vi "CP Profile selection_MS.vi"(8 "Signal Tag AZ":string[](array[string]), 11 "Long Signal Profile Table A":string[][](table) caption="Long Singla Profile Table") -> (3 "CP selected IDX":T1)   [LabVIEW 2018]
panel:
  out "M_MxRight_No":string[](array[string])
  out "M_RRead_Seq":string[](array[string])
  out "S# [n]":string[](array[string])
  out "L# [n]":string[](array[string])
  out "MSeq_ENo":string[](array[string])
  out "MSeq_SNo":string[](array[string])
  out "Later Seq":string[](array[string])
  out "Seq":string[](array[string])
  out "Front Seq":string[](array[string])
  out "Seq ENo":string[](array[string])
  out "Seq SNo":string[](array[string])
  out "Mx Right Read Seq":string[](array[string])
  out "Direction":string[](array[string])
  out "Assinged Sequence":string[](array[string])
  out "S CP IDX End [n]":string[](array[string])
  out "S CP IDX Start [n]":string[](array[string])
  out "サイズ":i32
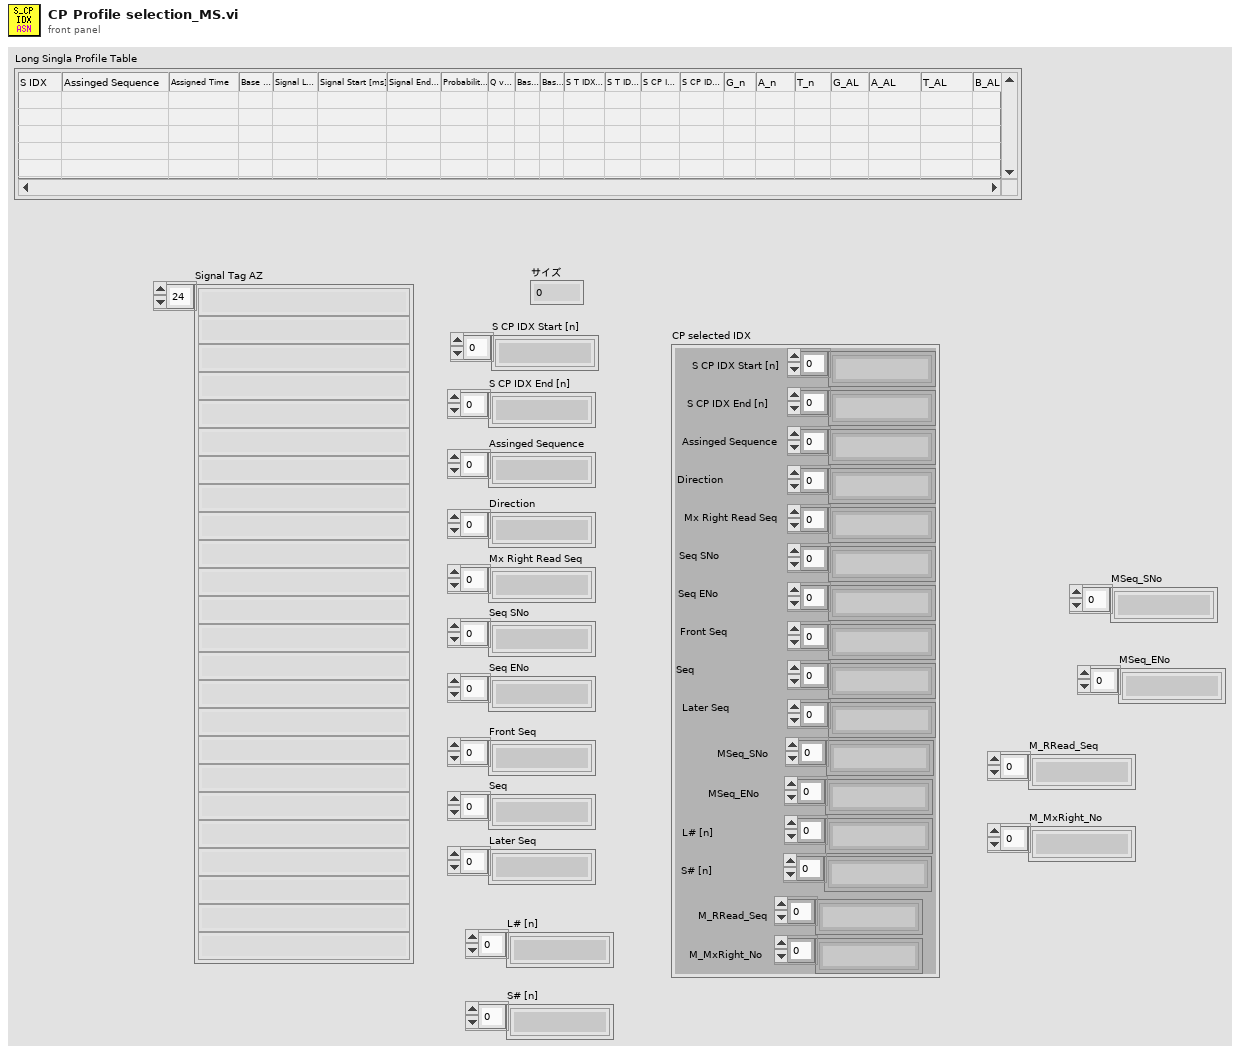
[diagram p1: front panel]
types:
  T1 = cluster{"S CP IDX Start [n]":string[], "S CP IDX End [n]":string[], "Assinged Sequence":string[], "Direction":string[], "Mx Right Read Seq":string[], "Seq SNo":string[], "Seq ENo":string[], "Front Seq":string[], "Seq":string[], "Later Seq":string[], "MSeq_SNo":string[], "MSeq_ENo":string[], "L# [n]":string[], "S# [n]":string[], "M_RRead_Seq":string[], "M_MxRight_No":string[]}
  T2 = cluster{string[], string[], string[], string[], string[], string[], string[], string[], string[], string[], string[], string[], string[], string[], string[], string[]}
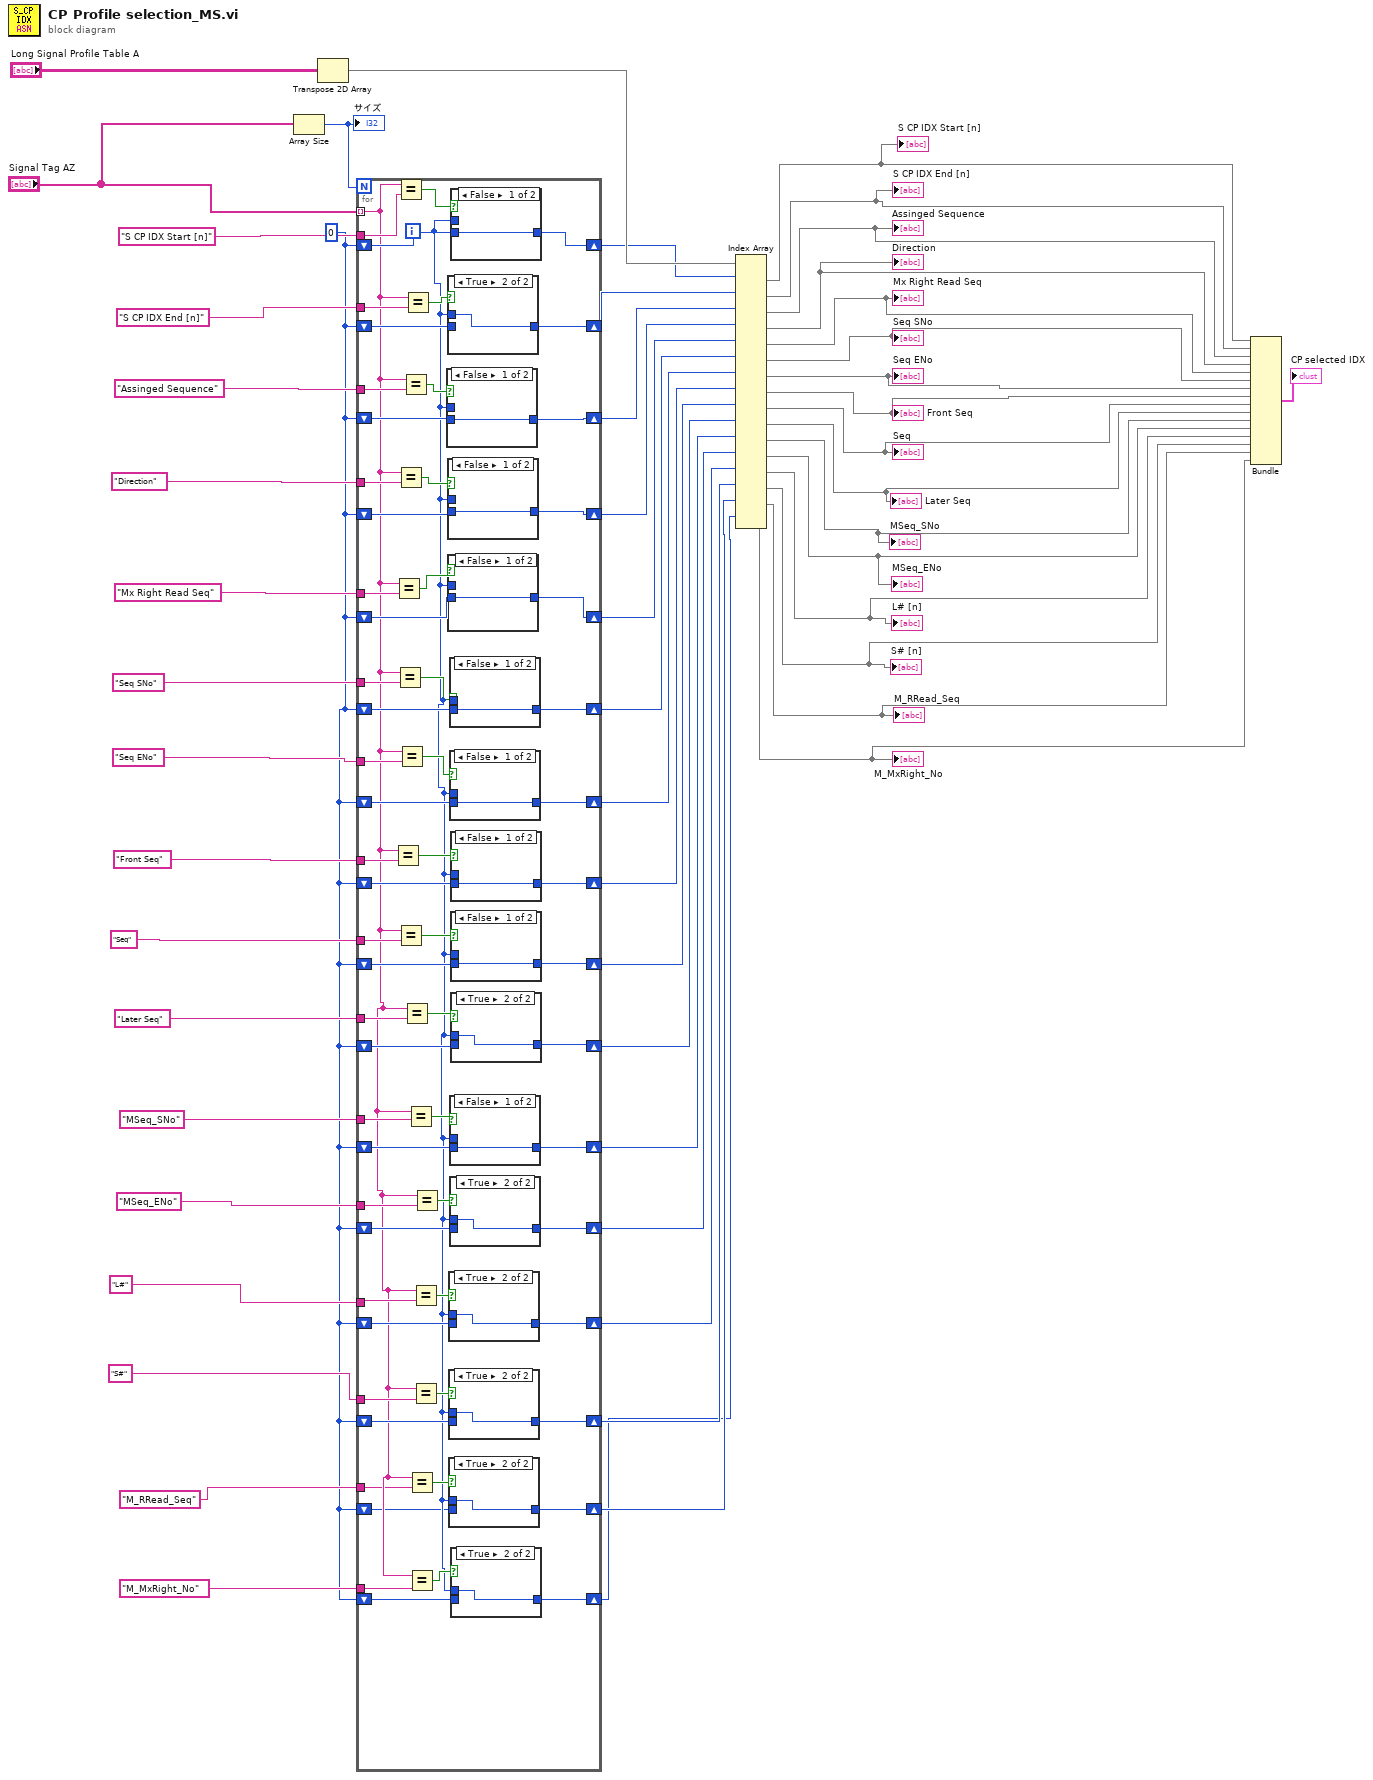
[diagram p0: block diagram]
diagram:
  w5 = 0
  n1 = Array Size(array="Signal Tag AZ") -> (size(s)=w54:i32)
  "サイズ" <- w54
  n2 = Transpose 2D Array(2D array="Long Signal Profile Table A") -> (transposed array=w53:string[][])
  n3 = for {
    N: w54 -> [_]
    tunnel: "Signal Tag AZ" -> [w64] mode=indexing
    tunnel: "S CP IDX Start [n]" -> [w120]
    shift-right: [w118] -> w51
    shift-left: w5 -> [w119]
    shift-right: [w115] -> w50
    shift-left: w5 -> [w116]
    shift-right: [w113] -> w49
    shift-left: w5 -> [w114]
    shift-right: [w111] -> w48
    shift-left: w5 -> [w112]
    shift-right: [w109] -> w47
    shift-left: w5 -> [w110]
    tunnel: "S CP IDX End [n]" -> [w107]
    tunnel: "Assinged Sequence" -> [w106]
    tunnel: "Direction" -> [w105]
    tunnel: "Mx Right Read Seq" -> [w104]
    shift-right: [w99] -> w38
    shift-left: w5 -> [w100]
    tunnel: "Seq SNo" -> [w97]
    tunnel: "Seq ENo" -> [w94]
    shift-right: [w95] -> w37
    shift-left: w5 -> [w96]
    shift-right: [w91] -> w33
    shift-left: w5 -> [w92]
    shift-right: [w89] -> w32
    shift-left: w5 -> [w90]
    shift-right: [w81] -> w31
    shift-left: w5 -> [w88]
    tunnel: "Front Seq" -> [w87]
    tunnel: "Seq" -> [w86]
    tunnel: "Later Seq" -> [w85]
    tunnel: "MSeq_SNo" -> [w80]
    tunnel: "MSeq_ENo" -> [w79]
    shift-right: [w78] -> w18
    shift-left: w5 -> [w77]
    shift-right: [w76] -> w17
    shift-left: w5 -> [w75]
    shift-right: [w71] -> w12
    shift-left: w5 -> [w69]
    tunnel: "L#" -> [w70]
    shift-right: [w67] -> w11
    shift-left: w5 -> [w65]
    tunnel: "S#" -> [w66]
    tunnel: "M_RRead_Seq" -> [w63]
    tunnel: "M_MxRight_No" -> [w61]
    shift-right: [w59] -> w4
    shift-left: w5 -> [w56]
    shift-right: [w57] -> w3
    shift-left: w5 -> [w55]
    i -> [w58]
    n4 = Equal?(x=w64, y=w87) -> (x = y?=w84:bool)
    n5 = Equal?(x=w64, y=w104) -> (x = y?=w101:bool)
    n6 = Equal?(x=w64, y=w97) -> (x = y?=w98:bool)
    n7 = Equal?(x=w64, y=w120) -> (x = y?=w117:bool)
    n8 = Equal?(x=w64, y=w105) -> (x = y?=w102:bool)
    n9 = Equal?(x=w64, y=w86) -> (x = y?=w83:bool)
    n10 = Equal?(x=w64, y=w94) -> (x = y?=w93:bool)
    n11 = Equal?(x=w64, y=w106) -> (x = y?=w103:bool)
    n12 = Equal?(x=w64, y=w85) -> (x = y?=w82:bool)
    n13 = Equal?(x=w64, y=w107) -> (x = y?=w108:bool)
    n14 = Equal?(x=w64, y=w80) -> (x = y?=w74:bool)
    n15 = Equal?(x=w64, y=w63) -> (x = y?=w62:bool)
    n16 = Equal?(x=w64, y=w61) -> (x = y?=w60:bool)
    n17 = Equal?(x=w64, y=w70) -> (x = y?=w72:bool)
    n18 = Equal?(x=w64, y=w66) -> (x = y?=w68:bool)
    n19 = Equal?(x=w64, y=w79) -> (x = y?=w73:bool)
    n20 = case shown="False" w103 {
      tunnel: w58 -> [_ w148]
      tunnel: [w147 w148] -> w113
      tunnel: w114 -> [w147 _]
      frame False {
      }
      frame True {
      }
    }
    n21 = case shown="True" w108 {
      tunnel: w58 -> [_ w150]
      tunnel: [w149 w150] -> w115
      tunnel: w116 -> [w149 _]
      frame False {
      }
      frame True {
      }
    }
    n22 = case shown="False" w102 {
      tunnel: w58 -> [_ w146]
      tunnel: [w145 w146] -> w111
      tunnel: w112 -> [w145 _]
      frame False {
      }
      frame True {
      }
    }
    n23 = case shown="False" w101 {
      tunnel: w58 -> [_ w144]
      tunnel: [w143 w144] -> w109
      tunnel: w110 -> [w143 _]
      frame False {
      }
      frame True {
      }
    }
    n24 = case shown="True" w72 {
      tunnel: w58 -> [_ w128]
      tunnel: [w127 w128] -> w71
      tunnel: w69 -> [w127 _]
      frame False {
      }
      frame True {
      }
    }
    n25 = case shown="True" w68 {
      tunnel: w58 -> [_ w126]
      tunnel: [w125 w126] -> w67
      tunnel: w65 -> [w125 _]
      frame False {
      }
      frame True {
      }
    }
    n26 = case shown="True" w62 {
      tunnel: w58 -> [_ w124]
      tunnel: [w123 w124] -> w59
      tunnel: w56 -> [w123 _]
      frame False {
      }
      frame True {
      }
    }
    n27 = case shown="False" w98 {
      tunnel: w58 -> [_ w142]
      tunnel: [w141 w142] -> w99
      tunnel: w100 -> [w141 _]
      frame False {
      }
      frame True {
      }
    }
    n28 = case shown="False" w93 {
      tunnel: w58 -> [_ w140]
      tunnel: [w139 w140] -> w95
      tunnel: w96 -> [w139 _]
      frame False {
      }
      frame True {
      }
    }
    n29 = case shown="False" w74 {
      tunnel: w58 -> [_ w132]
      tunnel: [w131 w132] -> w78
      tunnel: w77 -> [w131 _]
      frame False {
      }
      frame True {
      }
    }
    n30 = case shown="True" w73 {
      tunnel: w58 -> [_ w130]
      tunnel: [w129 w130] -> w76
      tunnel: w75 -> [w129 _]
      frame False {
      }
      frame True {
      }
    }
    n31 = case shown="False" w117 {
      tunnel: w58 -> [_ w152]
      tunnel: [w151 w152] -> w118
      tunnel: w119 -> [w151 _]
      frame False {
      }
      frame True {
      }
    }
    n32 = case shown="False" w84 {
      tunnel: w58 -> [_ w138]
      tunnel: [w137 w138] -> w91
      tunnel: w92 -> [w137 _]
      frame False {
      }
      frame True {
      }
    }
    n33 = case shown="False" w83 {
      tunnel: w58 -> [_ w136]
      tunnel: [w135 w136] -> w89
      tunnel: w90 -> [w135 _]
      frame False {
      }
      frame True {
      }
    }
    n34 = case shown="True" w82 {
      tunnel: w58 -> [_ w134]
      tunnel: [w133 w134] -> w81
      tunnel: w88 -> [w133 _]
      frame False {
      }
      frame True {
      }
    }
    n35 = case shown="True" w60 {
      tunnel: w58 -> [_ w122]
      tunnel: [w121 w122] -> w57
      tunnel: w55 -> [w121 _]
      frame False {
      }
      frame True {
      }
    }
  }
  n36 = Index Array(array=w53, index (row) #1=w51, index (row) #2=w50, index (row) #3=w49, index (row) #4=w48, index (row) #5=w47, index (row) #6=w38, index (row) #7=w37, index (row) #8=w33, index (row) #9=w32, index (row) #10=w31, index (row) #11=w18, index (row) #12=w17, index (row) #13=w12, index (row) #14=w11, index (row) #15=w4, index (row) #16=w3) -> (element #1=w30:string[], element #2=w10:string[], element #3=w29:string[], element #4=w28:string[], element #5=w27:string[], element #6=w26:string[], element #7=w25:string[], element #8=w24:string[], element #9=w23:string[], element #10=w22:string[], element #11=w16:string[], element #12=w15:string[], element #13=w9:string[], element #14=w8:string[], element #15=w2:string[], element #16=w1:string[])  [unwired: 16 in]
  "S CP IDX Start [n]" <- w30
  "S CP IDX End [n]" <- w10
  "Assinged Sequence" <- w29
  "Direction" <- w28
  "Mx Right Read Seq" <- w27
  "Seq SNo" <- w26
  "Seq ENo" <- w25
  "Front Seq" <- w24
  "Seq" <- w23
  "Later Seq" <- w22
  "MSeq_SNo" <- w16
  "MSeq_ENo" <- w15
  "L# [n]" <- w9
  "S# [n]" <- w8
  "M_RRead_Seq" <- w2
  "M_MxRight_No" <- w1
  n37 = Bundle(w30, w10, w29, w28, w27, w26, w25, w24, w23, w22, w16, w15, w9, w8, w2, w1) -> (→"CP selected IDX":T2)  [unwired: 1 in]
